vi "Run All Tests.vi"   [LabVIEW 2019, in "RemoteControl.ZMQ.Tests.lvclass"]
uses:
  RemoteControl.ZMQ.Tests.lvclass
  <vilib>/addons/_JKI Toolkits/Caraya/classes/Test/Test.lvclass
  src/ZMQ.ContextManager/ZMQ.ContextManager.lvlib
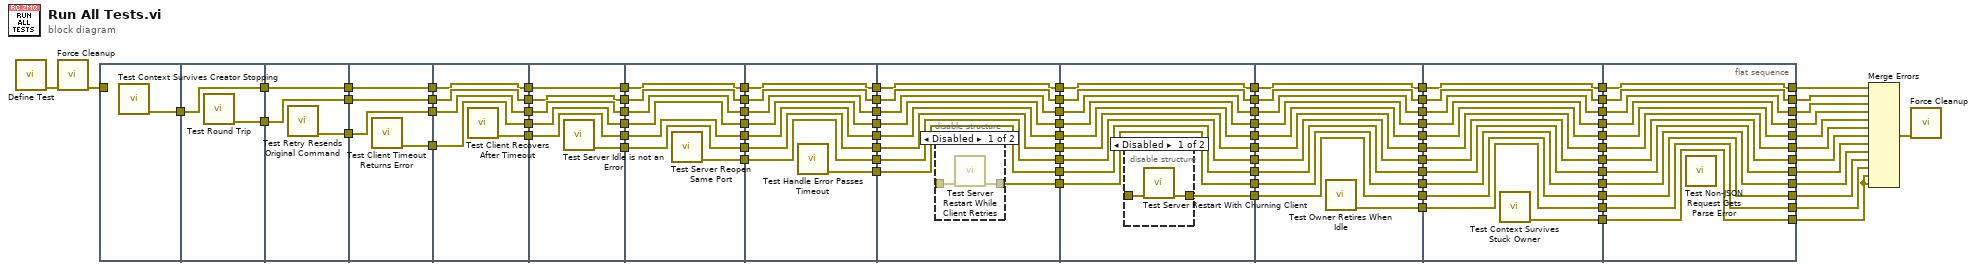
[diagram p0: block diagram]
diagram:
  n1 = call <vilib>:"Define Test.vi"() -> ("error out"=w40:errorcluster)  [unwired: 10 in, 1 out]
  n2 = call "Force Cleanup.vi"("error in"=w40) -> ("error out"=w20:errorcluster)  [unwired: 9 in, 1 out]
  n3 = flat-sequence {
    tunnel: [w94] -> w60
    tunnel: w20 -> [_]
    tunnel: [w96] -> w69
    tunnel: w60 -> [w95]
    tunnel: [w95] -> w59
    tunnel: [w99] -> w77
    tunnel: w69 -> [w98]
    tunnel: [w98] -> w68
    tunnel: w59 -> [w97]
    tunnel: [w97] -> w58
    tunnel: w77 -> [w103]
    tunnel: [w103] -> w76
    tunnel: w68 -> [w102]
    tunnel: [w102] -> w67
    tunnel: w58 -> [w101]
    tunnel: [w101] -> w57
    tunnel: [w100] -> w18
    tunnel: [w108] -> w83
    tunnel: w76 -> [w107]
    tunnel: [w107] -> w75
    tunnel: w67 -> [w106]
    tunnel: [w106] -> w66
    tunnel: w57 -> [w105]
    tunnel: [w105] -> w56
    tunnel: w18 -> [w104]
    tunnel: [w104] -> w17
    tunnel: w83 -> [w114]
    tunnel: [w114] -> w82
    tunnel: w75 -> [w113]
    tunnel: [w113] -> w74
    tunnel: w66 -> [w112]
    tunnel: [w112] -> w65
    tunnel: w56 -> [w111]
    tunnel: [w111] -> w55
    tunnel: w17 -> [w110]
    tunnel: [w110] -> w16
    tunnel: [w109] -> w8
    tunnel: [w121] -> w87
    tunnel: w82 -> [w120]
    tunnel: [w120] -> w81
    tunnel: w74 -> [w119]
    tunnel: [w119] -> w73
    tunnel: w65 -> [w118]
    tunnel: [w118] -> w64
    tunnel: w55 -> [w117]
    tunnel: [w117] -> w54
    tunnel: w16 -> [w116]
    tunnel: [w116] -> w15
    tunnel: w8 -> [w115]
    tunnel: [w115] -> w7
    tunnel: [w129] -> w90
    tunnel: w87 -> [w128]
    tunnel: [w128] -> w86
    tunnel: w81 -> [w127]
    tunnel: [w127] -> w80
    tunnel: w73 -> [w126]
    tunnel: [w126] -> w72
    tunnel: w64 -> [w125]
    tunnel: [w125] -> w63
    tunnel: w54 -> [w124]
    tunnel: [w124] -> w53
    tunnel: w15 -> [w123]
    tunnel: [w123] -> w14
    tunnel: w7 -> [w122]
    tunnel: [w122] -> w6
    tunnel: [w138] -> w92
    tunnel: w90 -> [w137]
    tunnel: [w137] -> w89
    tunnel: w86 -> [w136]
    tunnel: [w136] -> w85
    tunnel: w80 -> [w135]
    tunnel: [w135] -> w79
    tunnel: w72 -> [w134]
    tunnel: [w134] -> w71
    tunnel: w63 -> [w133]
    tunnel: [w133] -> w62
    tunnel: w53 -> [w132]
    tunnel: [w132] -> w52
    tunnel: w14 -> [w131]
    tunnel: [w131] -> w13
    tunnel: w6 -> [w130]
    tunnel: [w130] -> w5
    tunnel: w92 -> [w149]
    tunnel: w89 -> [w148]
    tunnel: w85 -> [w147]
    tunnel: w79 -> [w146]
    tunnel: w71 -> [w145]
    tunnel: w62 -> [w144]
    tunnel: w52 -> [w143]
    tunnel: [w150] -> w49
    tunnel: [w149] -> w48
    tunnel: [w148] -> w47
    tunnel: [w147] -> w46
    tunnel: [w146] -> w45
    tunnel: [w145] -> w44
    tunnel: [w144] -> w43
    tunnel: [w143] -> w42
    tunnel: w13 -> [w142]
    tunnel: [w142] -> w12
    tunnel: w5 -> [w141]
    tunnel: [w141] -> w4
    tunnel: w49 -> [w163]
    tunnel: w48 -> [w162]
    tunnel: w47 -> [w161]
    tunnel: w46 -> [w160]
    tunnel: w45 -> [w159]
    tunnel: w44 -> [w158]
    tunnel: w43 -> [w157]
    tunnel: w42 -> [w156]
    tunnel: [w163] -> w39
    tunnel: [w162] -> w38
    tunnel: [w161] -> w37
    tunnel: [w160] -> w36
    tunnel: [w159] -> w35
    tunnel: [w158] -> w34
    tunnel: [w157] -> w33
    tunnel: [w156] -> w32
    tunnel: [w155] -> w31
    tunnel: w12 -> [w154]
    tunnel: [w154] -> w11
    tunnel: w4 -> [w153]
    tunnel: [w153] -> w3
    tunnel: w39 -> [w175]
    tunnel: w38 -> [w174]
    tunnel: w37 -> [w173]
    tunnel: w36 -> [w172]
    tunnel: w35 -> [w171]
    tunnel: w34 -> [w170]
    tunnel: w33 -> [w169]
    tunnel: w32 -> [w168]
    tunnel: w31 -> [w167]
    tunnel: [w175] -> w30
    tunnel: [w174] -> w29
    tunnel: [w173] -> w28
    tunnel: [w172] -> w27
    tunnel: [w171] -> w26
    tunnel: [w170] -> w25
    tunnel: [w169] -> w24
    tunnel: [w168] -> w23
    tunnel: [w167] -> w22
    tunnel: [w166] -> w21
    tunnel: w11 -> [w165]
    tunnel: [w165] -> w10
    tunnel: w3 -> [w164]
    tunnel: [w164] -> w2
    tunnel: [w178] -> w19
    tunnel: [w179] -> w41
    tunnel: [w180] -> w51
    tunnel: [w181] -> w61
    tunnel: [w182] -> w70
    tunnel: [w183] -> w78
    tunnel: [w184] -> w84
    tunnel: [w185] -> w88
    tunnel: [w186] -> w91
    tunnel: [w187] -> w93
    tunnel: w30 -> [w187]
    tunnel: w29 -> [w186]
    tunnel: w28 -> [w185]
    tunnel: w27 -> [w184]
    tunnel: w26 -> [w183]
    tunnel: w25 -> [w182]
    tunnel: w24 -> [w181]
    tunnel: w23 -> [w180]
    tunnel: w22 -> [w179]
    tunnel: w21 -> [w178]
    tunnel: w10 -> [w177]
    tunnel: [w177] -> w9
    tunnel: w2 -> [w176]
    tunnel: [w176] -> w1
    frame #0 {
      n4 = call "Test Context Survives Creator Stopping.vi"() -> ("error out"=w94:errorcluster)  [unwired: 11 in]
    }
    frame #1 {
      n5 = call "Test Round Trip.vi"() -> ("error out"=w96:errorcluster)  [unwired: 11 in]
    }
    frame #2 {
      n6 = call "Test Retry Resends Original Command.vi"() -> ("error out"=w99:errorcluster)  [unwired: 11 in]
    }
    frame #3 {
      n7 = call "Test Client Timeout Returns Error.vi"() -> ("error out"=w100:errorcluster)  [unwired: 11 in]
    }
    frame #4 {
      n8 = call "Test Client Recovers After Timeout.vi"() -> ("error out"=w108:errorcluster)  [unwired: 11 in]
    }
    frame #5 {
      n9 = call "Test Server Idle is not an Error.vi"() -> ("error out"=w109:errorcluster)  [unwired: 11 in]
    }
    frame #6 {
      n10 = call "Test Server Reopen Same Port.vi"() -> ("error out"=w121:errorcluster)  [unwired: 11 in]
    }
    frame #7 {
      n11 = call "Test Handle Error Passes Timeout.vi"() -> ("error out"=w129:errorcluster)  [unwired: 11 in]
    }
    frame #8 {
      n12 = disable-structure shown="Disabled" {
        disable-tunnel: _ -> [w140 _]
        disable-tunnel: [w139 _] -> w138
        frame Disabled {
          n13 = call "Test Server Restart While Client Retries.vi"("error in (no error)"=w140) -> ("error out"=w139:errorcluster)  [unwired: 10 in]
        }
        frame Enabled {
        }
      }
    }
    frame #9 {
      n14 = disable-structure shown="Disabled" {
        disable-tunnel: _ -> [w152 _]
        disable-tunnel: [w151 _] -> w150
        frame Disabled {
          n15 = call "Test Server Restart With Churning Client.vi"("error in (no error)"=w152) -> ("error out"=w151:errorcluster)  [unwired: 10 in]
        }
        frame Enabled {
        }
      }
    }
    frame #10 {
      n16 = call "Test Owner Retires When Idle.vi"() -> ("error out"=w155:errorcluster)  [unwired: 11 in]
    }
    frame #11 {
      n17 = call "Test Context Survives Stuck Owner.vi"() -> ("error out"=w166:errorcluster)  [unwired: 11 in]
    }
    frame #12 {
      n18 = call "Test Non-JSON Request Gets Parse Error.vi"() -> ()  [unwired: 11 in, 1 out]
    }
  }
  n19 = Merge Errors(w51, w61, w70, w9, w78, w1, w84, w88, w91, w93, w41, w19, w19) -> (w50:errorcluster)
  n20 = call "Force Cleanup.vi"("error in"=w50) -> ()  [unwired: 9 in, 2 out]
